vi "GetContextHelpInfo.vi"(0 "reference in":refnum<class "DQMHModuleNode.lvclass">, 1 "MousePos":T1 {"y" format="%.2f"; "x" format="%.2f"}, 5 "error in (no error)":errorcluster) -> (14 "reference out":refnum<class "DQMHModuleNode.lvclass">, 15 "ContextHelpInfoExist":bool, 16 "ContextHelpInfo":variant, 19 "error out":errorcluster)   [LabVIEW 2020, in "DQMHModuleNode.lvclass"]
doc: "GetContextHelpInfo"
uses:
  <resource>/Framework/Providers/Open_GDS/UML/DQMHModuleNode_class/DQMHModuleNode.lvclass
  C:/Program Files (x86)/National Instruments/LabVIEW 2020/resource/Framework/Providers/Open_GDS/UML/RectangularNode_class/RectangularNode.lvclass
  <resource>/Framework/Providers/Open_GDS/UML/General/Point/Point Point2D.ctl
  <resource>/Framework/Providers/Open_GDS/UML/MultiLineString_class/MultiLineString.lvclass
  <resource>/Framework/Providers/Open_GDS/ClassProviders/Provider_BaseClassInterface/ClassReader_class/ClassReader.lvclass
  <resource>/Framework/Providers/Open_GDS/UML/RectangularNode_class/RectangularNode.lvclass
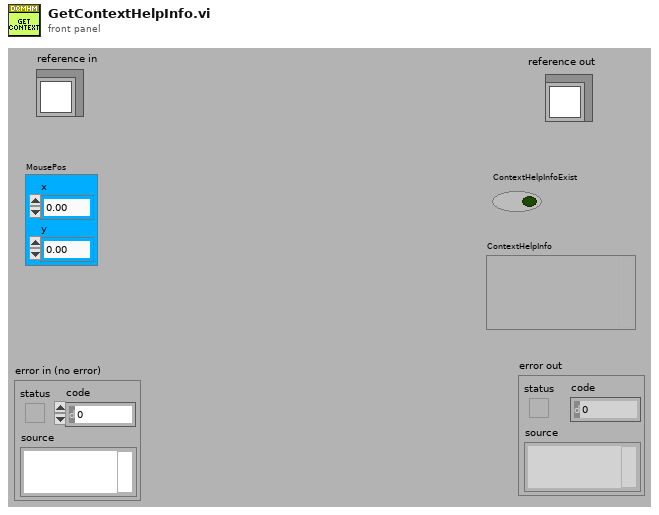
[diagram p1: front panel]
types:
  T1 = typedef "Point Point2D.ctl" = cluster{"x":dbl, "y":dbl}
  T2 = typedef "DQMHModuleNode.lvclass/ObjectAttributes.ctl" = cluster{"DescriptionHeight":dbl, "InternalDataHeight":dbl, "EventsHeight":dbl, "Name":refnum<class "MultiLineString.lvclass">, "Description":refnum<class "MultiLineString.lvclass">, "InternalData":refnum<class "MultiLineString.lvclass">, "Events":refnum<class "MultiLineString.lvclass">, "showDescription":bool, "showInternalData":bool, "showEvents":bool, "DEFAULT_ROUNDING":i32, "DEFAULT_WIDTH":i32, "DEFAULT_HEIGHT":i32, "ClassPath":path, "Template":string, "Icon":u8[][]}
  T3 = typedef "RectangularNode.lvclass/ObjectAttributes.ctl" = cluster{"bounds":T4}
  T4 = typedef "Rectangle Rectangle2D.ctl" = cluster{"x":dbl, "y":dbl, "width":dbl, "height":dbl}
  T5 = cluster{"text":string, "empty picture":picture, "Description":string}
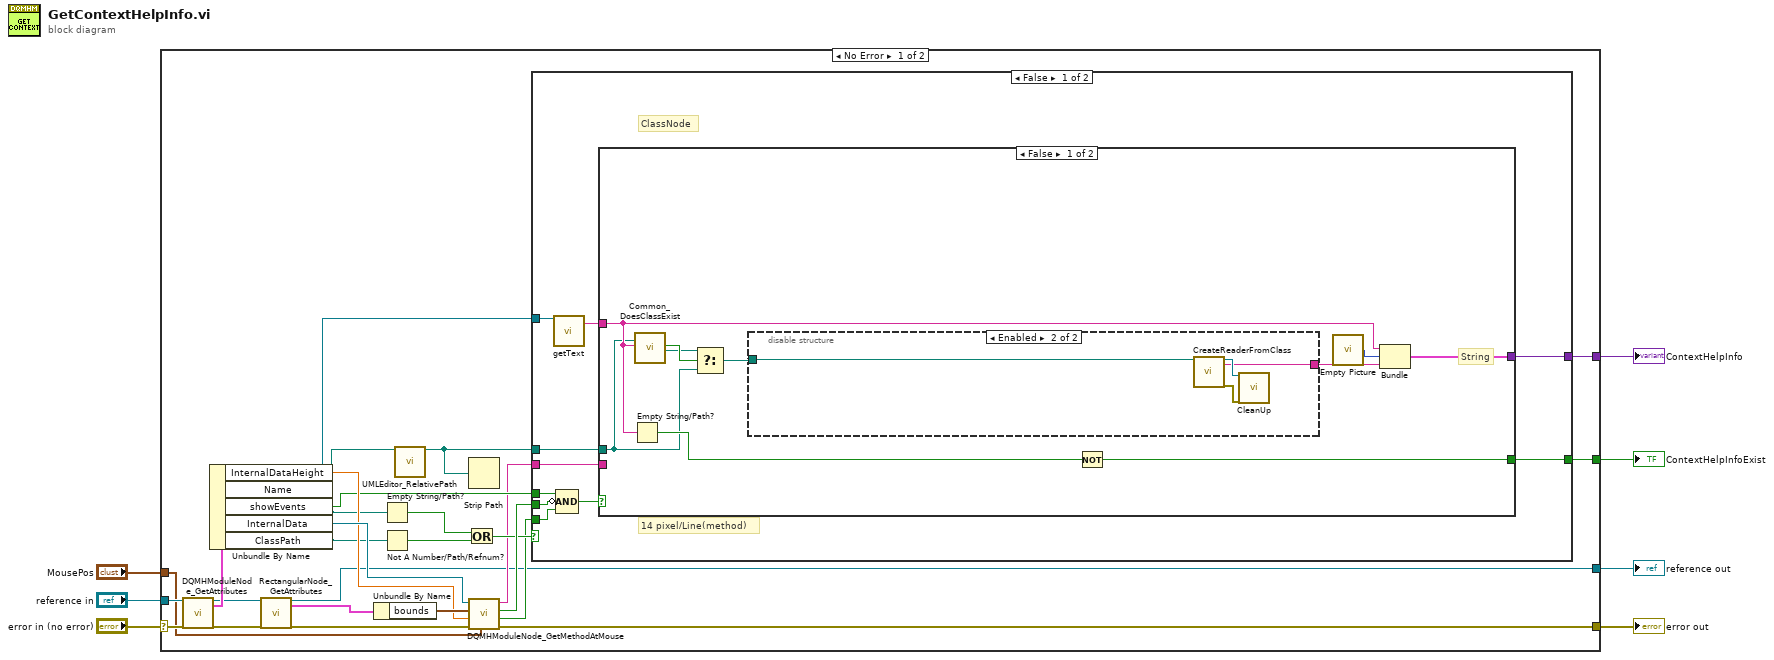
[diagram p0: block diagram]
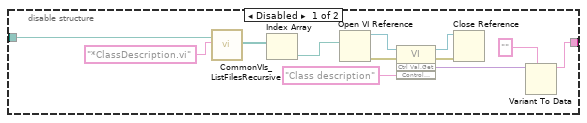
[diagram p2: hidden frame]
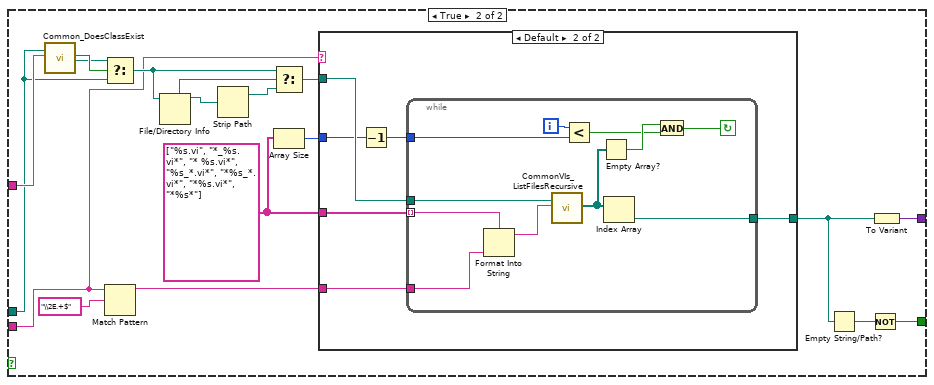
[diagram p3: hidden frame]
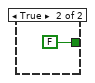
[diagram p5: hidden frame]
diagram:
  n1 = case shown="No Error" "error in (no error)" {
    selector: "error in (no error)" -> [w32 w105]
    tunnel: "reference in" -> [w31 w106]
    tunnel: [w28 w105] -> w5
    tunnel: [w9 w106] -> w4
    tunnel: "MousePos" -> [w29 _]
    tunnel: [w27 _] -> w2
    tunnel: [w26 _] -> w1
    frame No Error {
      n2 = call <resource>:"DQMHModuleNode_GetAttributes.vi"("reference in"=w31, "error in (no error)"=w32) -> ("reference out"=w12:refnum<class "DQMHModuleNode.lvclass">, "Data"=w13:T2, "error out"=w11:errorcluster)  [unwired: 1 in, 14 out]
      n3 = Unbundle By Name(w13) -> ("InternalDataHeight"=w24:dbl, "Name"=w21:refnum<class "MultiLineString.lvclass">, "showEvents"=w22:bool, "InternalData"=w30:refnum<class "MultiLineString.lvclass">, "ClassPath"=w16:path)
      n4 = call <resource>:"RectangularNode_GetAttributes.vi"("reference in"=w12, "error in (no error)"=w11) -> ("reference out"=w9:refnum<class "DQMHModuleNode.lvclass">, "Data"=w8:T3, "error out"=w10:errorcluster)  [unwired: 14 in, 1 out]
      n5 = Unbundle By Name(w8) -> ("bounds"=w25:T4)
      n6 = Empty String/Path?(string/path=w16) -> (empty?=w20:bool)
      n7 = Not A Number/Path/Refnum?(number/path/refnum=w16) -> (NaN/Path/Refnum?=w19:bool)
      n8 = call <resource>:"UMLEditor_RelativePath.vi"("Path In"=w16) -> ("ConvertToAbsolutePath(If possible)"=w17:path)  [unwired: 1 in, 17 out]
      n9 = Or(x=w20, y=w19) -> (x .or. y?=w18:bool)
      n10 = Strip Path(path=w17) -> ()  [unwired: 2 out]
      n11 = call <resource>:"DQMHModuleNode_GetMethodAtMouse.vi"("MousePos"=w29, "error in"=w10, "botHeight"=w24, "bounds"=w25, "reference in"=w30) -> ("error out"=w28:errorcluster, "MethodSelected"=w15:bool, "NoMmethodsExists"=w23:bool, "MEthodName"=w14:string)  [unwired: 1 in]
      n12 = case shown="False" w18 {
        tunnel: [w42 _] -> w27
        tunnel: [w41 FALSE] -> w26
        tunnel: w23 -> [w40 _]
        tunnel: w22 -> [w38 _]
        tunnel: w21 -> [w37 _]
        tunnel: w17 -> [w39 _]
        tunnel: w15 -> [w36 _]
        tunnel: w14 -> [w35 _]
        frame False {
          # "ClassNode"
          # "14 pixel/Line(method)"
          n13 = call-dynamic "getText.vi"("reference"=w37) -> ("text"=w33:string)  [unwired: 1 in, 17 out]
          n14 = Compound Arithmetic op=AND(w38, invert w40, w36) -> (w34:bool)
          n15 = case shown="False" w34 {
            tunnel: w39 -> [w44 w83]
            tunnel: [w50 w85] -> w42
            tunnel: [w48 w78] -> w41
            tunnel: w33 -> [w45 w84]
            tunnel: w35 -> [_ w69]
            frame False {
              # "String"
              n16 = Empty String/Path?(string/path=w45) -> (empty?=w49:bool)
              n17 = call <resource>:"Common_DoesClassExist.vi"("ClassPath"=w44, "ClassName"=w45) -> ("llb-class"=w47:bool, "llb/LvCLass-Path"=w46:path)  [unwired: 16 out]
              n18 = Select(t=w46, s=w47, f=w44) -> (s? t:f=w43:path)
              n19 = disable-structure shown="Enabled" {
                disable-tunnel: [w54 w65] -> w51
                disable-tunnel: w43 -> [w53 w66]
                frame Disabled {
                  n20 = call <resource>:"CommonVIs_ListFilesRecursive.vi"("directory path"=w53, "FileSearchPattern"="*ClassDescription.vi") -> ("Files"=w64:path[])  [unwired: 14 in, 3 out]
                  n21 = Index Array(array=w64) -> (element=w62:path)  [unwired: 1 in]
                  n22 = Open VI Reference(vi path=w62) -> (vi reference=w60:refnum<vi>, error out=w61:errorcluster)  [unwired: 5 in]
                  n23 = invoke class="VI" method="Ctrl Val.Get"(reference=w60, error in=w61, "Control Name"="Class description") -> (reference out=w58:refnum<vi>, error out=w57:errorcluster, "Get Control Value Variant"=w56:variant)  [unwired: 1 in, 1 out]
                  n24 = Close Reference(reference=w58, error in (no error)=w57) -> ()  [unwired: 1 out]
                  n25 = Variant To Data(type="", Variant=w56) -> (data=w54:string)  [unwired: 1 in, 1 out]
                }
                frame Enabled {
                  n26 = call <resource>:"CreateReaderFromClass.vi"("ClassPath/LvClassRef"=w66) -> ("ClassReader"=w67:refnum<class "ClassReader.lvclass">, "Description"=w65:string, "error out"=w68:errorcluster)  [unwired: 1 in, 15 out]
                  n27 = call-dynamic "CleanUp.vi"("reference in"=w67, "error in (no error)"=w68) -> ()  [unwired: 18 out]
                }
              }
              n28 = Not(x=w49) -> (.not. x?=w48:bool)
              n29 = call "Empty Picture"() -> ("empty picture"=w52:picture)
              n30 = Bundle("text"=w45, "empty picture"=w52, "Description"=w51) -> (w50:T5)  [unwired: 1 out]
            }
            frame True {
              w74 = string[] ["%s.vi", "*_%s.vi*", "* %s.vi*", "%s_*.vi*", "*%s_*.vi*", "*%s.vi*", "*%s*"]
              n31 = call <resource>:"Common_DoesClassExist.vi"("ClassPath"=w83, "ClassName"=w84) -> ("llb-class"=w82:bool, "llb/LvCLass-Path"=w81:path)  [unwired: 16 out]
              n32 = Select(t=w81, s=w82, f=w83) -> (s? t:f=w70:path)
              n33 = Match Pattern(string=w69, regular expression="\\2E.+$") -> (before substring=w75:string)  [unwired: 4 out]
              n34 = File/Directory Info(path=w70) -> (path out=w72:path, directory=w77:bool)  [unwired: 1 in, 5 out]
              n35 = Strip Path(path=w72) -> (stripped path=w71:path)  [unwired: 1 out]
              n36 = Select(t=w70, s=w77, f=w71) -> (s? t:f=w76:path)
              n37 = Array Size(array=w74) -> (size(s)=w73:i32)
              n38 = case shown="Default" w69 {
                tunnel: [_ w89] -> w80
                tunnel: w76 -> [_ w92]
                tunnel: w74 -> [_ w91]
                tunnel: w75 -> [_ w90]
                tunnel: w73 -> [_ w88]
                frame "" {
                }
                frame Default {
                  n39 = Decrement(x=w88) -> (x-1=w87:i32)
                  n40 = while {
                    tunnel: w92 -> [w103]
                    tunnel: w91 -> [w102] mode=indexing
                    tunnel: w90 -> [w101]
                    tunnel: [w100] -> w89
                    tunnel: w87 -> [w96]
                    i -> [w97]
                    stop <- w93 continue-if-true
                    n41 = Format Into String(format string=w102, w101) -> (resulting string=w98:string)  [unwired: 2 in, 1 out]
                    n42 = call <resource>:"CommonVIs_ListFilesRecursive.vi"("directory path"=w103, "FileSearchPattern"=w98) -> ("Files"=w99:path[])  [unwired: 4 in, 13 out]
                    n43 = Less?(x=w97, y=w96) -> (x < y?=w94:bool)
                    n44 = Empty Array?(array=w99) -> (empty?=w95:bool)
                    n45 = Index Array(array=w99) -> (element=w100:path)  [unwired: 1 in]
                    n46 = And(x=w95, y=w94) -> (x .and. y?=w93:bool)
                  }
                }
              }
              n47 = Empty String/Path?(string/path=w80) -> (empty?=w79:bool)
              n48 = Not(x=w79) -> (.not. x?=w78:bool)
              n49 = To Variant(anything=w80) -> (Variant=w85:variant)
            }
          }
        }
        frame True {
        }
      }
    }
    frame Error {
    }
  }
  "reference out" <- w4
  "error out" <- w5
  "ContextHelpInfo" <- w2
  "ContextHelpInfoExist" <- w1
